vi "Util_GetTime.vi"(8 "error in (no error)":errorcluster, 11 "Pass_Through_Time":dbl=-1.0 format="%33.4f") -> (0 "error out":errorcluster, 2 "FPGA_Time_MicroSeconds":u64 format="%.0g", 3 "FPGA_Time_Seconds":dbl format="%33.4f")   [LabVIEW 2019, in "Trajectory_Library.lvlib"]
doc: "This subVI returns the continuously running elapsed time in seconds. \n\nOn the RoboRIO this reads the high resolution FPGA time. The resolution, not accuracy, of the FPGA timer is 1 microsecond. The normal FPGA clock register (32 bits) rolls over approximately every 71 minutes. To significantly extend the rollover time,, this routine reads both the high and low FPGA clock registers. High/low register turnover read sequencing is dealt with by reading the high register twice, once before and once after the low register. If the values are different, the read is repeated to assure consistency between the high and low values. On a PC the standard operating system timer with 1 millisecond resolution is used. \n\nNotes:\n-------\n- On the RoboRIO this routine takes approximately 2.1 microseconds to execute. When both words of the FPGA clock have to be read the routine takes approximately 4.2 microseconds. This occurs once every 71 minutes when the routine determines that the low word has rolled over. The WPI read FPGA clock routine takes approxmately 2.1 microseconds. The difference can be attributed to this routine reading to extra words from the FPGA. Each FPGA read takes approximately 1 microsecond. \n\n- Set a conditional complilation variable TRAJLIB_USEOSTIME and set it to a value of 1 to force this routine to read the RoboRIO operating system time instead of the FPGA time. This will have 1 millisecond resolution. This routine executes faster, approx 1 microsecond.\n\n - On the RoboRIO there is some drift between the FPGA and operating system clocks. The drift isn't consistent, but appears to be approximately 20 milliseconds / hour. This isn't enough to be of concern.\n\n\nInput parameters:\n - PassThroughTime -- double float -- If wired and the value is > 0 then this time is passed through and the FPGA time is not read. Allows calling functions to use a single time instant if desired.\n - Input Error -- Input error cluster\n\nReturns:\n - FPGA_Time_Seconds -- double float -- Elapsed time in seconds.\n - FPGA_Time_Microseconds -- Uint64 -- Elapsed time in microseconds (This can be used as an input to the Network Table routines to sychnronize times.)\n - Output Error -- Output error cluster. An error will be returned if there are problems reading the FPGA or of the FPGA clock high register changes twice while reading the value.\n\nCustom Errors:\n - 8020 -- The upper FPGA time register changed during both attempts to read the FPGA time values. The returned time may not be valid."
uses:
  Trajectory_Library.lvlib
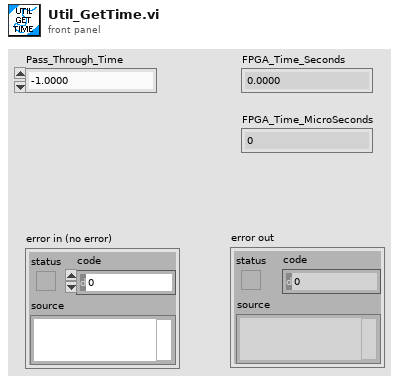
[diagram p1: front panel]
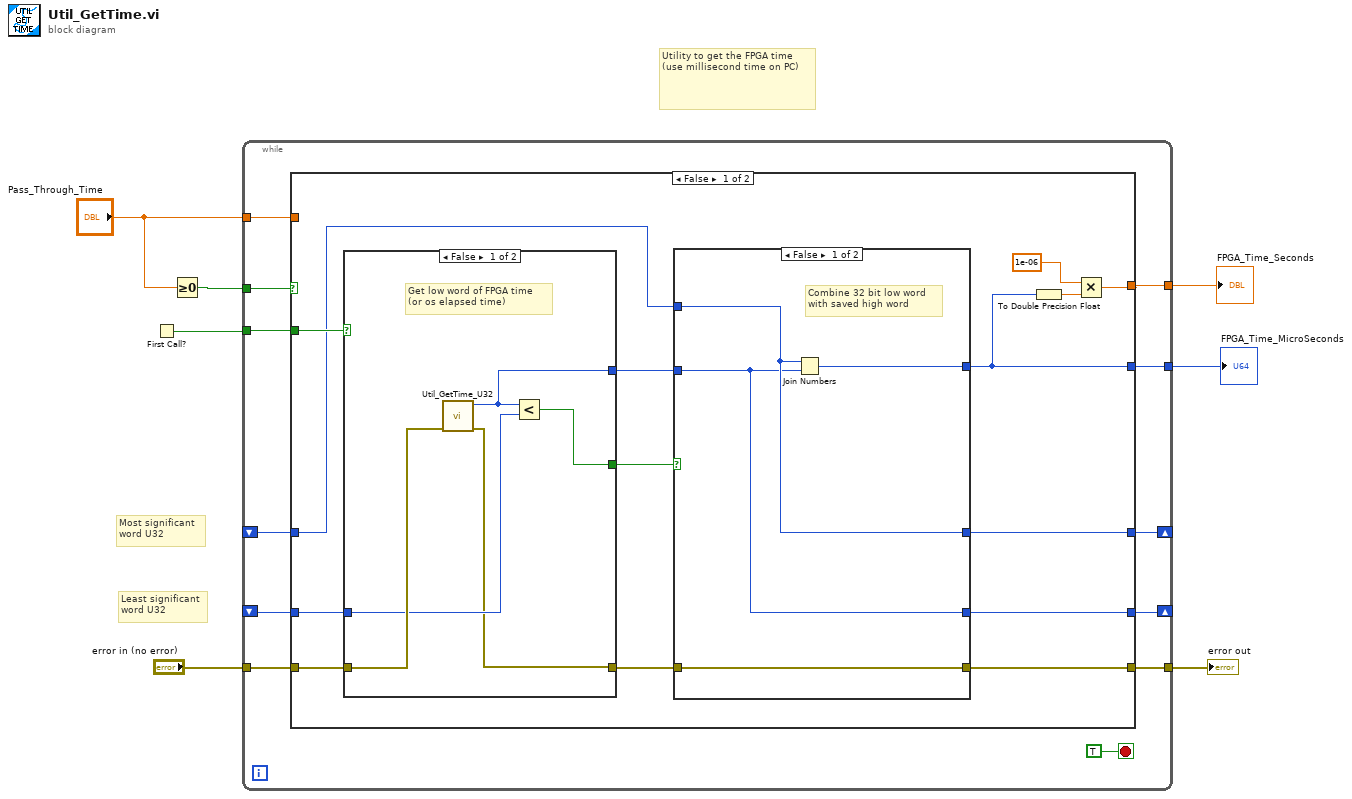
[diagram p0: block diagram]
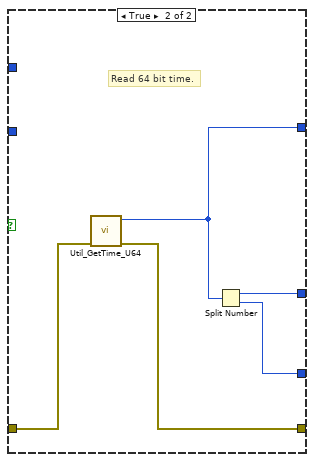
[diagram p2: hidden frame]
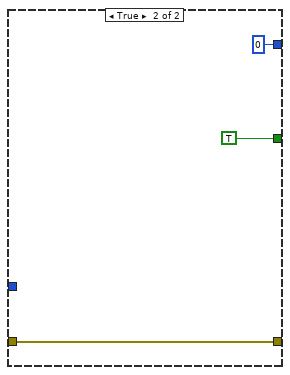
[diagram p3: hidden frame]
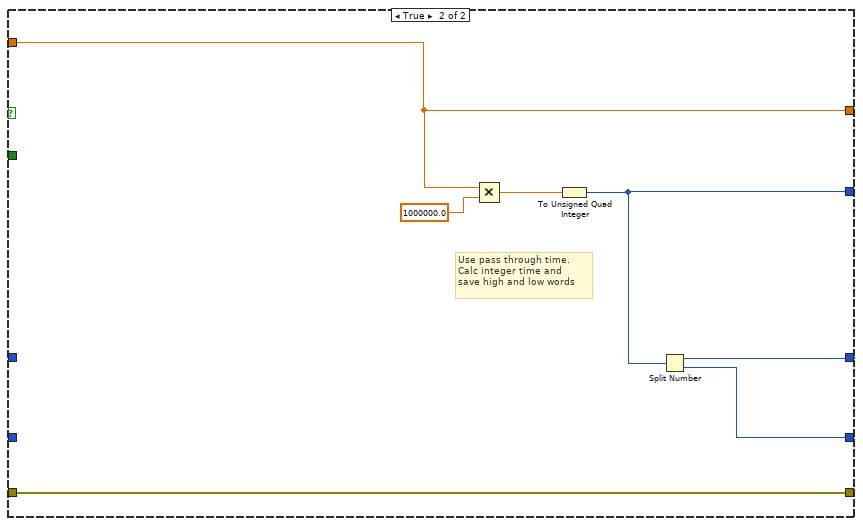
[diagram p4: hidden frame]
diagram:
  # "Least significant\nword U32"
  # "Most significant\nword U32"
  # "Utility to get the FPGA time\n(use millisecond time on PC)"
  n1 = First Call?() -> (First Call?: T/F=w1:bool)
  n2 = Greater Or Equal To 0?(x="Pass_Through_Time") -> (x >= 0?=w7:bool)
  n3 = while {
    shift-right: [w12] -> _
    shift-left: _ -> [w8]
    tunnel: w7 -> [w18]
    tunnel: "error in (no error)" -> [w17]
    tunnel: "Pass_Through_Time" -> [w16]
    tunnel: [w15] -> w4
    tunnel: [w14] -> w3
    tunnel: [w13] -> w2
    tunnel: w1 -> [w11]
    shift-right: [w10] -> _
    shift-left: _ -> [w9]
    stop <- TRUE stop-if-true
    n4 = case shown="False" w18 {
      tunnel: w17 -> [w32 w54]
      tunnel: w16 -> [_ w55]
      tunnel: [w21 w55] -> w15
      tunnel: [w20 w53] -> w14
      tunnel: [w30 w54] -> w13
      tunnel: [w27 w52] -> w12
      tunnel: w11 -> [w33 _]
      tunnel: [w28 w51] -> w10
      tunnel: w9 -> [w25 _]
      tunnel: w8 -> [w24 _]
      frame False {
        n5 = case shown="False" w33 {
          tunnel: w32 -> [w47 w49]
          tunnel: [w44 TRUE] -> w31
          tunnel: [w43 w49] -> w29
          tunnel: [w46 u32 0 ("FPGA_Time_LowWord_MicroSeconds")] -> w26
          tunnel: w25 -> [w45 _]
          frame False {
            # "Get low word of FPGA time\n(or os elapsed time)"
            n6 = call "Util_GetTime_U32.vi"("error in (no error)"=w47) -> ("error out"=w43:errorcluster, "FPGA_Time_LowWord_MicroSeconds"=w46:u32)  [unwired: 9 in]
            n7 = Less?(x=w46, y=w45) -> (x < y?=w44:bool)
          }
          frame True {
          }
        }
        n8 = case shown="False" w31 {
          tunnel: [w37 w42] -> w30
          tunnel: w29 -> [w37 w41]
          tunnel: [w34 w40] -> w28
          tunnel: [w35 w39] -> w27
          tunnel: [w36 w38] -> w20
          tunnel: w26 -> [w34 _]
          tunnel: w24 -> [w35 _]
          frame False {
            # "Combine 32 bit low word\nwith saved high word"
            n9 = Join Numbers(hi=w35, lo=w34) -> ((hi.lo)=w36:u64)
          }
          frame True {
            # "Read 64 bit time."
            n10 = call "Util_GetTime_U64.vi"("error in (no error)"=w41) -> ("error out"=w42:errorcluster, "FPGA_Time_MicroSeconds"=w38:u64)  [unwired: 9 in]
            n11 = Split Number(x=w38) -> (hi(x)=w39:u32, lo(x)=w40:u32)
          }
        }
        n12 = To Double Precision Float(number=w20) -> (double precision float=w23:dbl)
        n13 = Multiply(x=1e-06, y=w23) -> (x*y=w21:dbl)
      }
      frame True {
        # "Use pass through time.    \nCalc integer time and \nsave high and low words"
        n14 = Multiply(x=w55, y=1000000.0) -> (x*y=w56:dbl)
        n15 = To Unsigned Quad Integer(1:w56) -> (0:w53:u64)
        n16 = Split Number(x=w53) -> (hi(x)=w52:u32, lo(x)=w51:u32)
      }
    }
  }
  "FPGA_Time_Seconds" <- w4
  "error out" <- w2
  "FPGA_Time_MicroSeconds" <- w3
